vi "Serial_Comunication.vi"(8 "Error_in":errorcluster, 9 "Timeout_ms":u32=3000, 10 "Command":string, 11 "VISA_resource_in":refnum<visa-resource-name>) -> (0 "Error_out":errorcluster, 2 "Response":string, 3 "VISA_resource_out":refnum<visa-resource-name>)   [LabVIEW 2026]
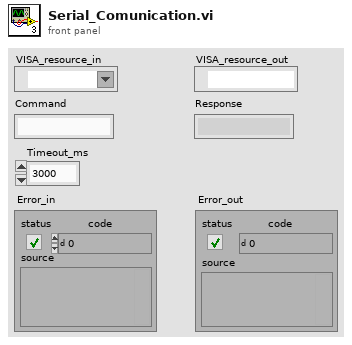
[diagram p1: front panel]
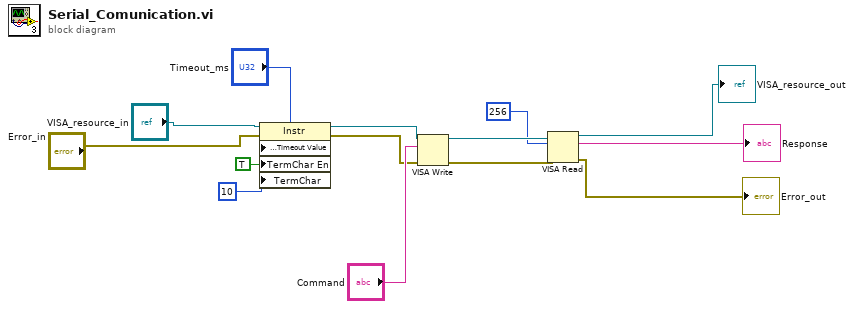
[diagram p0: block diagram]
diagram:
  n1 = property class="Instr"(reference="VISA_resource_in", error in="Error_in", "General Settings:Timeout Value"="Timeout_ms", "TermChar En"=TRUE ("Message Based Settings:Termination Character Enable"), "TermChar"=u8 10 ("Message Based Settings:Termination Character")) -> (reference out=w5:refnum<visa-resource-name>, error out=w3:errorcluster)
  n2 = VISA Write(VISA resource name=w5, write buffer="Command", error in (no error)=w3) -> (VISA resource name out=w14:refnum<visa-resource-name>, error out=w10:errorcluster)  [unwired: 1 out]
  n3 = VISA Read(VISA resource name=w14, byte count=u32 256, error in (no error)=w10) -> (VISA resource name out=→"VISA_resource_out":refnum<visa-resource-name>, read buffer=→"Response":string, error out=→"Error_out":errorcluster)  [unwired: 1 out]
